vi "RFH-add-Permittivity_from_calc.vi"() -> ()   [LabVIEW 2020, in "RFH-Reflection_File_Handler.lvlib"]
doc: "Run by hand: reads the files of a folder, computes the permittivity with the Bilinear method from the chosen air/open, DI water and salt water files at the given water temperature, and saves the results. The user picks the folder and the standard names."
uses:
  RFH-Reflection_File_Handler.lvlib
  Computation/RDC-Reflection_Data_Computation.lvlib
panel:
  in  "water Temp (25C) [10-40C]":dbl=22.5
  out "appended array":string[](array[string])
  in  "Cancel":bool
  in  "Continue":bool
  out "saltwater name":string
  out "DI-Water name":string
  out "Air/open name":string
  in  "File Path":path=path "C:/projects/Universitet/Master/data/autopermtest/lib"
  in  "Saltwater name":string="saltwater"
  in  "DI-water name":string="water"
  in  "Air/open name":string="air"
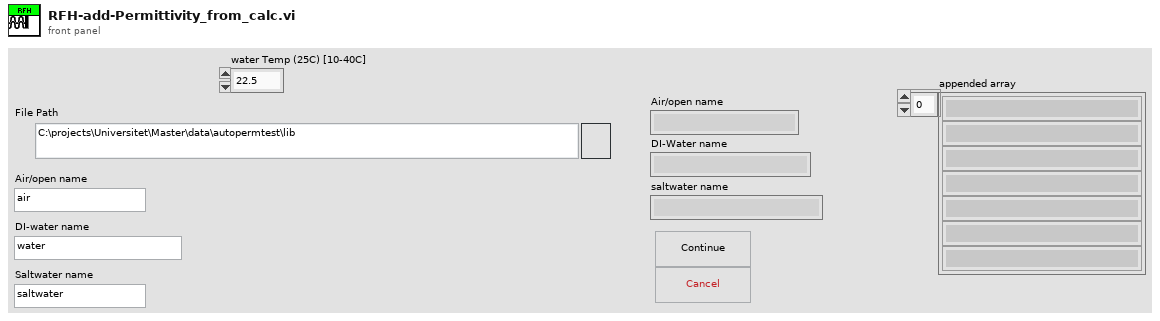
[diagram p1: front panel]
types:
  T1 = typedef "RFH-Reflection_File_Handler.lvlib/RFH-common_data_format.ctl" = cluster{"Frequency":dbl[], "Reflection'":dbl[], "Reflection''":dbl[], "Permativity'":dbl[], "Permativity''":dbl[], "Conductivity":dbl[], "Loss Tangent":dbl[], "Resistance":dbl[], "Reactance":dbl[]}
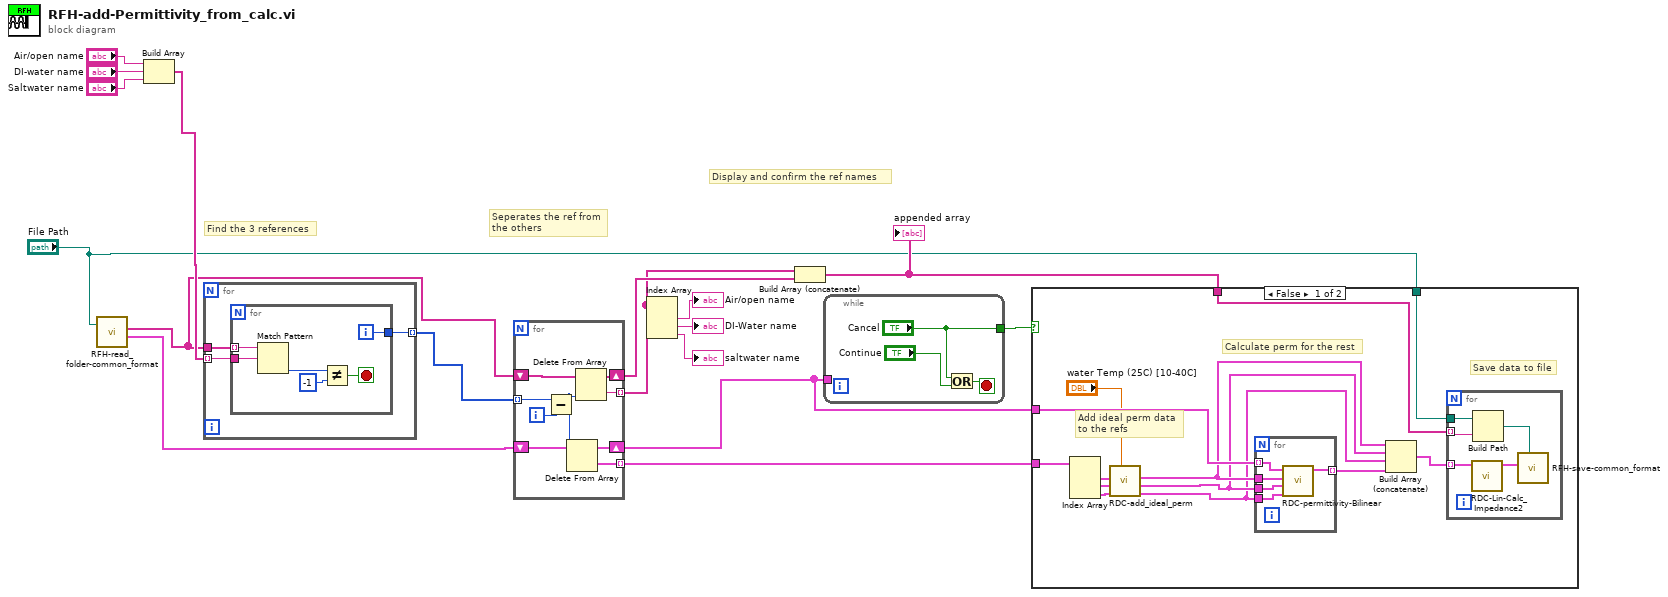
[diagram p0: block diagram]
diagram:
  # "Display and confirm the ref names"
  # "Seperates the ref from\nthe others"
  # "Find the 3 references"
  n1 = call "RFH-read_folder-common_format.vi"("File Path"="File Path") -> ("Data"=w8:T1[], "Names"=w12:string[])  [unwired: 8 in, 1 out]
  n2 = Build Array("Air/open name", "DI-water name", "Saltwater name") -> (w15:string[])
  n3 = for {
    tunnel: w12 -> [w19]
    tunnel: w15 -> [w20] mode=indexing
    tunnel: [w18] -> w13 mode=indexing
    n4 = for {
      tunnel: w20 -> [w25]
      tunnel: w19 -> [w26] mode=indexing
      tunnel: [w21] -> w18
      i -> [w21]
      stop <- w22 stop-if-true
      n5 = Match Pattern(string=w26, regular expression=w25) -> (offset past match=w24:i32)  [unwired: 1 in, 3 out]
      n6 = Not Equal?(x=w24, y=-1) -> (x != y?=w22:bool)
    }
  }
  n7 = for {
    tunnel: w13 -> [w34] mode=indexing
    shift-right: [w32] -> w4
    shift-left: w12 -> [w35]
    tunnel: [w31] -> w3 mode=indexing
    shift-right: [w29] -> w5
    shift-left: w8 -> [w30]
    tunnel: [w27] -> w6 mode=indexing
    i -> [w33]
    n8 = Subtract(x=w34, y=w33) -> (x-y=w28:i32)
    n9 = Delete From Array(array=w30, index=w28) -> (deleted portion=w27:T1, array with subset deleted=w29:T1[])  [unwired: 1 in]
    n10 = Delete From Array(array=w35, index=w28) -> (deleted portion=w31:string, array with subset deleted=w32:string[])  [unwired: 1 in]
  }
  n11 = Index Array(array=w3) -> (element #1=→"Air/open name":string, element #2=→"DI-Water name":string, element #3=→"saltwater name":string)  [unwired: 3 in]
  n12 = Build Array (concatenate)(w3, w4) -> (w2:string[])
  "appended array" <- w2
  n13 = while {
    tunnel: w5 -> [_]
    tunnel: ["Cancel"] -> w7
    stop <- w38 stop-if-true
    n14 = Or(x="Cancel", y="Continue") -> (x .or. y?=w38:bool)
  }
  n15 = case shown="False" w7 {
    tunnel: w6 -> [w46 _]
    tunnel: w5 -> [w48 _]
    tunnel: w2 -> [w44 _]
    tunnel: "File Path" -> [w45 _]
    frame False {
      # "Save data to file"
      # "Calculate perm for the rest"
      # "Add ideal perm data\nto the refs"
      n16 = Index Array(array=w46) -> (element #1=w51:T1, element #2=w50:T1, element #3=w49:T1)  [unwired: 3 in]
      n17 = call "RDC-add_ideal_perm.vi"("water Temp (25C) [10-40C]"="water Temp (25C) [10-40C]", "Salt Water"=w49, "DI-Water"=w50, "Open/Air"=w51) -> ("Salt Water out"=w40:T1, "DI-Water  out"=w41:T1, "Open/Air out"=w42:T1)  [unwired: 5 in]
      n18 = for {
        tunnel: w42 -> [w61]
        tunnel: w41 -> [w60]
        tunnel: w40 -> [w59]
        tunnel: w48 -> [w58] mode=indexing
        tunnel: [w57] -> w47 mode=indexing
        n19 = call "RDC-permittivity-Bilinear.vi"("Salt Water"=w59, "DI-Water"=w60, "Open/Air"=w61, "Common Format"=w58) -> ("Common Format out"=w57:T1)  [unwired: 7 in]
      }
      n20 = Build Array (concatenate)(w42, w41, w40, w47) -> (w43:T1[])
      n21 = for {
        tunnel: w45 -> [w56]
        tunnel: w44 -> [w55] mode=indexing
        tunnel: w43 -> [w53] mode=indexing
        n22 = call "RDC-Lin-Calc_Impedance2.vi"("input cluster"=w53) -> ("Output cluster"=w52:T1)  [unwired: 9 in, 1 out]
        n23 = Build Path(base path=w56, name or relative path=w55) -> (appended path=w54:path)
        n24 = call "RFH-save-common_format.vi"("file path (use dialog)"=w54, "Common Format"=w52) -> ()  [unwired: 9 in, 1 out]
      }
    }
    frame True {
    }
  }
